vi "UI - By List.vi"(5 "Term (Methods)":string="Methods", 7 "Msg Chain":string, 8 "error in (no error)":errorcluster {"code" format="Error %.0f"}, 10 "UI Docs":refnum<class "GUI Documentation.lvclass">[](array[class]), 11 "VIDoc Printer - Confluence In":refnum<class "VIDoc Printer - Confluence.lvclass">) -> (0 "error out":errorcluster {"code" format="Error %.0f"}, 3 "VIDoc Printer - Confluence Out":refnum<class "VIDoc Printer - Confluence.lvclass">)   [LabVIEW 2023, in "VIDoc Printer - Confluence.lvlib" / "VIDoc Printer - Confluence.lvclass"]
uses:
  VIDoc Printer - Confluence.lvclass
  <vilib>/DMC/VIDoc/Framework/Parsing/GUI Documentation/GUI Documentation.lvclass
  Confluence Formatting/Types/Format Combo Box.ctl
  <vilib>/DMC/VIDoc/Framework/Printer/VIDoc Printer.lvclass/VIDoc Printer.ctl
  VIDoc Printer - Confluence.lvclass/VIDoc Printer - Confluence.ctl
  <vilib>/DMC/VIDoc/Framework/Parsing/GUI Documentation/GUI Documentation.lvclass/GUI Documentation.ctl
  Types/VI Method Types.ctl
  <vilib>/DMC/VIDoc/Framework/Printer/Accessors/Get VI Settings - List Detail Level.vi
  <vilib>/DMC/VIDoc/Framework/Parsing/GUI Documentation/Get VI Info.vi
  <vilib>/DMC/VIDoc/Framework/Printer/Accessors/Get Formatting Settings - Bookmark Options.vi
  Accessors/Get Sortable Tables.vi
  Accessors/Get Temporary Image Directory+.vi
  Accessors/Get VI By List Expand.vi
  <vilib>/Utility/libraryn.llb/Create Directory Recursive.vi
  Confluence Formatting/Confluence Formatting.lvlib
  <vilib>/DMC/VIDoc/Framework/Printer/VIDoc Printer.lvclass
  <vilib>/DMC/VIDoc/Framework/UI Interaction/Interface/UI Interaction.lvclass
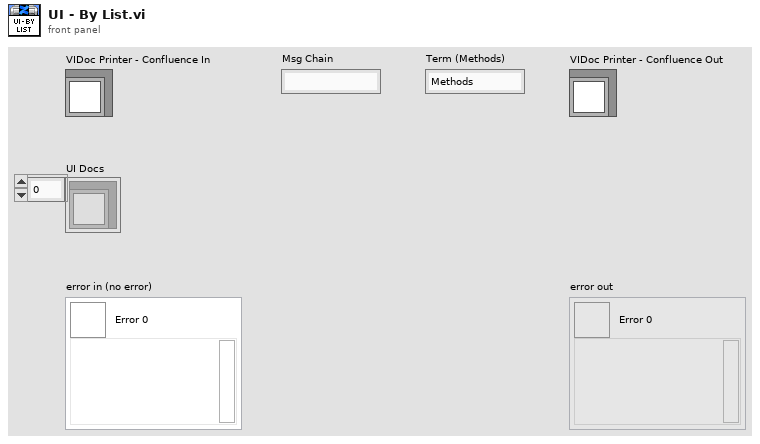
[diagram p1: front panel]
types:
  T1 = typedef "Confluence Formatting.lvlib/Format Combo Box.ctl" = string
  T2 = typedef "VIDoc Printer.lvlib/Printer Settings.lvclass/VI Settings.ctl" = cluster{"Memory":bool, "By Folder":bool, "By Tree":bool, "By List":bool, "Methods":bool, "Method Options":cluster{"Front Panels":bool, "Options":bool, "Controls":bool}, "List Detail Level":T3, "Methods Detail Level":T3, "Controls Detail Level":T3}
  T3 = typedef "VIDoc Printer.lvlib/Printer Settings.lvclass/Detail Level Enum.ctl" = enum16{"None", "Minimal", "Standard", "Full"}
  T4 = typedef "VIDoc Printer.lvlib/Printer Settings.lvclass/Bookmark Options.ctl" = cluster{"Bookmarks as New Line in VI Descriptions":bool, "Unique Bookmark Tags Only":bool, "Include Tag and Text":bool}
  T5 = typedef "VIDoc Printer - Confluence.lvlib/VIDoc Printer - Confluence.lvclass/VI Method Types.ctl" = enum16{"Library", "Class", "Interface", "LLB", "UI", "List"}
  T6 = typedef "VIDoc Parsing.lvlib/Method Spec Cluster.ctl" = cluster{"VI Type Ext":T7, "Name":string, "Path":path, "Get Conpane Image":T8, "Description":string, "Get Library Access Scope":enum32{"invalid scope", "public", "private", "protected", "community"}, "Dispatch":T9, "ContainsCompiledCode":bool, "Exec.IsReentrant":bool, "Exec.ReentrancyType":enum16{"Share clones between instances", "Preallocate clone for each instance"}, "ExecInlining":bool, "ExecInlineIfPossible":bool, "Auto Err Handling":bool, "CodeComplexity":sgl, "Bookmark Tags":string[], "Control VI Type":enum32{"not a control VI", "control", "typedef", "strict typedef"}, "Controls":T10[], "VI Type":enum32{"invalid VI type", "Standard VI", "Control VI", "Global VI", "Polymorphic VI", "Configuration VI", "SubSystem", "Facade VI", "Method VI", "Statechart Diagram VI"}, "Minimum Size":T12, "Front Panel Window:Title":string, "Front Panel Window:Behavior":enum32{"Invalid", "Default", "Floating", "Floating/Auto-Hide", "Modal"}, "Front Panel Window:Closeable":bool, "Must Override":bool, "Must Use Parent Implementation":bool, "VI Icon":T8, "Front Panel":T8, "History:Revision Number":u32, "Metrics:Total Data Size":u32, "Execution:Allow Debugging":bool, "Execution:Preferred Exec System":enum32{"invalid execution system", "user interface", "standard", "instrument i/o", "data acquisition", "other 1", "other 2", "same as caller"}, "Execution:Priority":enum32{"invalid priority", "background priority", "normal priority", "above normal priority", "high priority", "time critical priority", "subroutine"}, "BM Tag Text":string[], "Block Diagram":T8, "Structure Tree":T13[]}
  T7 = typedef "VIDoc Parsing.lvlib/VI Type Extended Enum.ctl" = enum16{"Unknown", "Class Method", "Class Accessor Get", "Class Accessor Set", "Class Control", "Library Method", "Library Control", "VI", "Control"}
  T8 = typedef "imagedata.ctl" = cluster{"image type":i32, "image depth":i32, "image":u8[], "mask":u8[], "colors":u32[], "Rectangle":cluster{"left":i16, "top":i16, "right":i16, "bottom":i16}}
  T9 = typedef "VIDoc Parsing.lvlib/Class Dispatch Type Enum.ctl" = enum16{"None", "Static", "Dynamic"}
  T10 = typedef "VIDoc Parsing.lvlib/Controls Info Cluster.ctl" = cluster{"Name":string, "Description":string, "Data Type":string, "Tip Strip":string, "UID":i32, "Image Data":T8, "ToggleKeyBind":T11, "Raw Label":string, "Raw Caption":string}
  T11 = typedef "LVKeyTypeDef.ctl" = cluster{"Focus":bool, "Control":bool, "Shift":bool, "Key":string}
  T12 = typedef "LVPointTypeDef.ctl" = cluster{"Horizontal":i16, "Vertical":i16}
  T13 = typedef "VIDoc Parsing.lvlib/Structure Reporter.lvlib/Tree Cluster.ctl" = cluster{"Object Class Name":string, "Labels":string[], "Child Tag":string, "Item Indent":i32, "Child Only?":bool, "Glyph Index":i32}
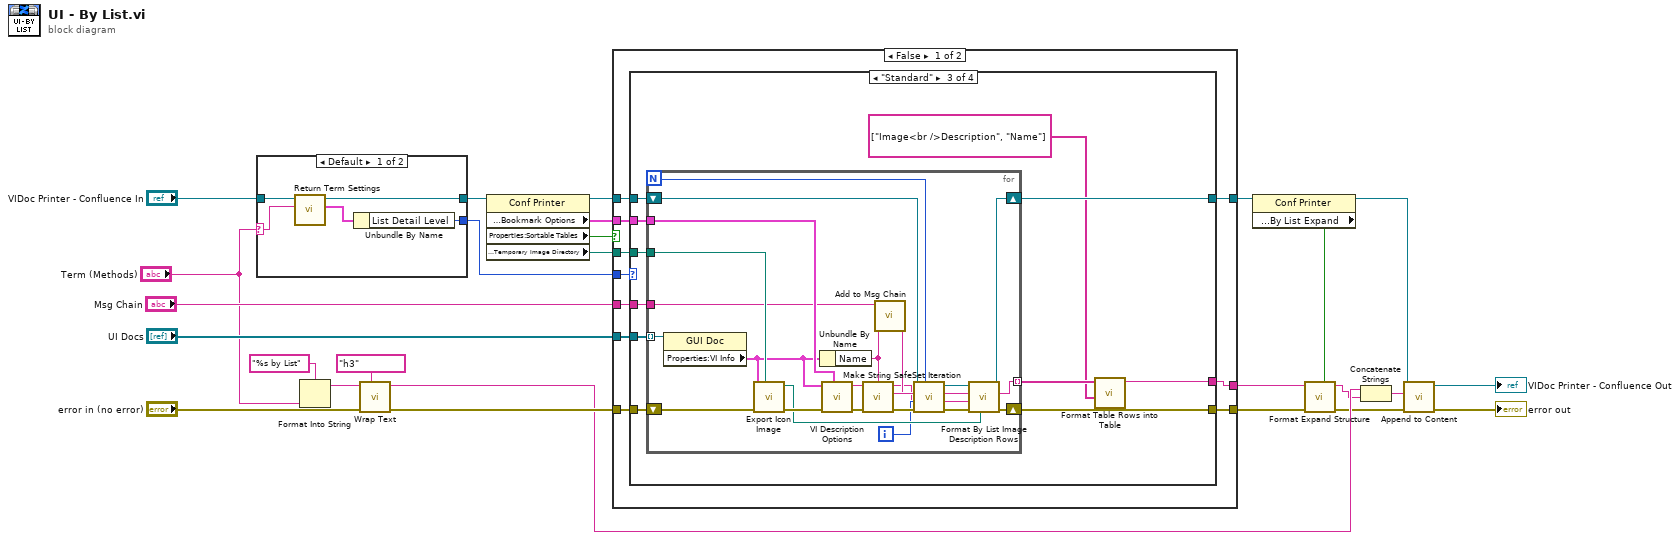
[diagram p0: block diagram]
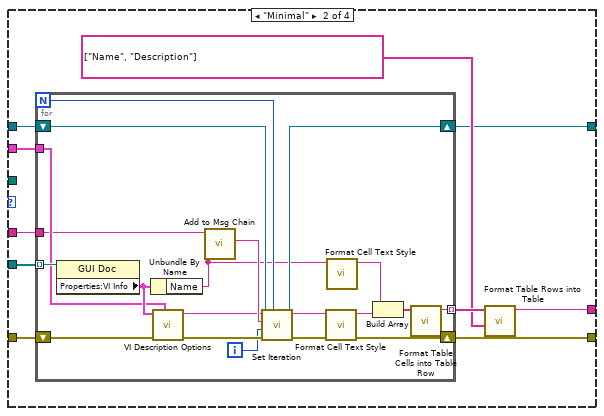
[diagram p3: hidden frame]
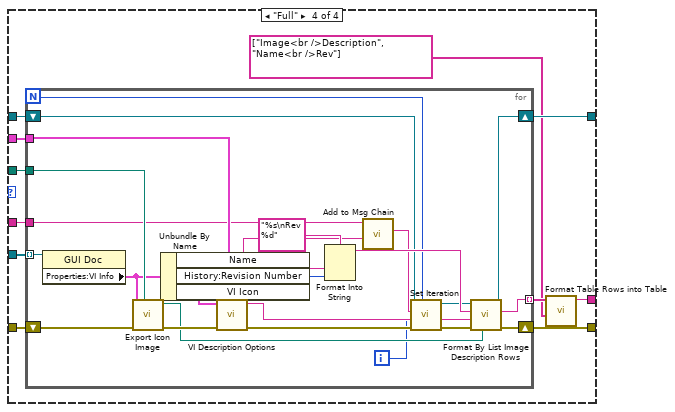
[diagram p4: hidden frame]
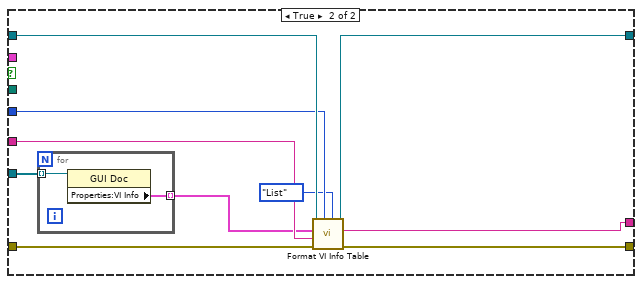
[diagram p5: hidden frame]
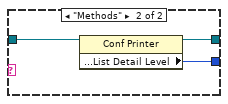
[diagram p6: hidden frame]
diagram:
  n1 = case shown="Default" "Term (Methods)" {
    selector: "Term (Methods)" -> [w29 _]
    tunnel: "VIDoc Printer - Confluence In" -> [w31 w34]
    tunnel: [w30 w33] -> w10
    tunnel: [w27 w32] -> w9
    frame Default {
      n2 = call <vilib>:"Return Term Settings.vi"("Term"=w29, "Printer in"=w31) -> ("Term Settings"=w28:T2, "Printer out"=w30:refnum<class "VIDoc Printer - Confluence.lvclass">)  [unwired: 6 in, 2 out]
      n3 = Unbundle By Name(w28) -> ("List Detail Level"=w27:T3)
    }
    frame "Methods" {
      n4 = property class="Conf Printer"(reference=w34) -> (reference out=w33:refnum<class "VIDoc Printer - Confluence.lvclass">, "Properties:Settings:VI Members:List Detail Level"=w32:T3)  [unwired: 1 in, 1 out]
    }
  }
  n5 = Format Into String(format string="%s by List", "Term (Methods)") -> (resulting string=w20:string)  [unwired: 2 in, 1 out]
  n6 = call "Wrap Text.vi"("Formatting"=T1 "h3", "Error in"="error in (no error)", "String"=w20) -> ("Error out"=w19:errorcluster, "Wrapped String"=w13:string)  [unwired: 7 in]
  n7 = property class="Conf Printer"(reference=w10) -> (reference out=w16:refnum<class "VIDoc Printer - Confluence.lvclass">, "Properties:Settings:Formatting Options:Bookmark Options"=w11:T4, "Properties:Sortable Tables"=w3:bool, "Properties:Temporary Image Directory"=w2:path)  [unwired: 1 in, 1 out]
  n8 = case shown="False" w3 {
    tunnel: w19 -> [w44 w150]
    tunnel: [w43 w149] -> w18
    tunnel: "UI Docs" -> [w42 w142]
    tunnel: w16 -> [w41 w147]
    tunnel: [w40 w146] -> w15
    tunnel: w2 -> [w39 _]
    tunnel: "Msg Chain" -> [w38 w143]
    tunnel: w11 -> [w37 _]
    tunnel: w9 -> [w36 w145]
    tunnel: [w35 w148] -> w7
    frame False {
      n9 = case shown="\"Standard\"" w36 {
        tunnel: w44 -> [w46 w54 w83 w115]
        tunnel: [w46 w51 w77 w109] -> w43
        tunnel: w42 -> [_ w56 w85 w117]
        tunnel: w37 -> [_ w55 w84 w116]
        tunnel: [_ w52 w79 w111] -> w35
        tunnel: w41 -> [w45 w49 w81 w113]
        tunnel: [w45 w48 w80 w112] -> w40
        tunnel: w39 -> [_ _ w82 w114]
        tunnel: w38 -> [_ w47 w75 w107]
        frame "None", Default {
        }
        frame "Minimal" {
          n10 = for {
            N -> [w64]
            tunnel: w56 -> [w74] mode=indexing
            tunnel: w55 -> [w72]
            shift-right: [w67] -> w51
            shift-left: w54 -> [w71]
            tunnel: [w69] -> w53 mode=indexing
            shift-right: [w65] -> w48
            shift-left: w49 -> [w66]
            tunnel: w47 -> [w62]
            i -> [w63]
            n11 = property class="GUI Doc"(reference=w74) -> ("Properties:VI Info"=w73:T6)  [unwired: 1 in, 2 out]
            n12 = Unbundle By Name(w73) -> ("Name"=w59:string)
            n13 = call <vilib>:"VI Description Options.vi"("Bookmark Options"=w72, "Error in"=w71, "VI Info"=w73) -> ("Error out"=w68:errorcluster, "Description"=w58:string)  [unwired: 7 in]
            n14 = call <vilib>:"Add to Msg Chain.vi"("New"=w59, "Msg Chain in"=w62) -> ("Msg Chain out"=w61:string)  [unwired: 9 in]
            n15 = call <vilib>:"Set Iteration.vi"("Progress Max"=w64, "error in (no error)"=w68, "Progress Value"=w63, "Message (No Message Update)"=w61, "VIDoc Printer In"=w66) -> ("error out"=w67:errorcluster, "VIDoc Printer Out"=w65:refnum<class "VIDoc Printer - Confluence.lvclass">)  [unwired: 4 in, 1 out]
            n16 = call "Format Cell Text Style.vi"("String"=w58) -> ("Formatted Text"=w57:string)  [unwired: 9 in, 1 out]
            n17 = call "Format Cell Text Style.vi"("String"=w59) -> ("Formatted Text"=w60:string)  [unwired: 9 in, 1 out]
            n18 = Build Array(w60, w57) -> (w70:string[])
            n19 = call "Format Table Cells into Table Row.vi"("Table Cells"=w70) -> ("Table Row Text"=w69:string)  [unwired: 10 in]
          }
          n20 = call "Format Table Rows into Table.vi"("Table Headers"=string[] ["Name", "Description"], "Table Rows"=w53) -> ("Table Text"=w52:string)  [unwired: 9 in]
        }
        frame "Standard" {
          n21 = for {
            N -> [w91]
            tunnel: w85 -> [w106] mode=indexing
            tunnel: w84 -> [w105]
            shift-right: [w100] -> w77
            shift-left: w83 -> [w103]
            tunnel: w82 -> [w104]
            shift-right: [w99] -> w80
            shift-left: w81 -> [w93]
            tunnel: [w96] -> w78 mode=indexing
            tunnel: w75 -> [w89]
            i -> [w90]
            n22 = property class="GUI Doc"(reference=w106) -> ("Properties:VI Info"=w101:T6)  [unwired: 1 in, 2 out]
            n23 = call <vilib>:"Export Icon Image.vi"("Temporary Image Directory"=w104, "Error in"=w103, "VI Info"=w101) -> ("Error out"=w102:errorcluster, "Image Path"=w97:path)  [unwired: 7 in]
            n24 = Unbundle By Name(w101) -> ("Name"=w88:string)
            n25 = call <vilib>:"VI Description Options.vi"("Bookmark Options"=w105, "Error in"=w102, "VI Info"=w101) -> ("Error out"=w95:errorcluster, "Description"=w98:string)  [unwired: 7 in]
            n26 = call "Make String Safe.vi"("Raw String"=w98) -> ("String out"=w86:string)  [unwired: 9 in, 1 out]
            n27 = call <vilib>:"Add to Msg Chain.vi"("New"=w88, "Msg Chain in"=w89) -> ("Msg Chain out"=w87:string)  [unwired: 9 in]
            n28 = call <vilib>:"Set Iteration.vi"("Progress Max"=w91, "error in (no error)"=w95, "Progress Value"=w90, "Message (No Message Update)"=w87, "VIDoc Printer In"=w93) -> ("error out"=w94:errorcluster, "VIDoc Printer Out"=w92:refnum<class "VIDoc Printer - Confluence.lvclass">)  [unwired: 4 in, 1 out]
            n29 = call "Format By List Image Description Rows.vi"("Image"=w97, "error in (no error)"=w94, "Description"=w86, "Name"=w88, "VIDoc Printer - Confluence In"=w92) -> ("error out"=w100:errorcluster, "Table Rows Text"=w96:string, "VIDoc Printer - Confluence Out"=w99:refnum<class "VIDoc Printer - Confluence.lvclass">)  [unwired: 3 in, 1 out]
          }
          n30 = call "Format Table Rows into Table.vi"("Table Headers"=string[] ["Image<br />Description", "Name"], "Table Rows"=w78) -> ("Table Text"=w79:string)  [unwired: 9 in]
        }
        frame "Full" {
          n31 = for {
            N -> [w122]
            tunnel: w117 -> [w140] mode=indexing
            tunnel: w116 -> [w139]
            shift-right: [w134] -> w109
            shift-left: w115 -> [w137]
            tunnel: w114 -> [w138]
            shift-right: [w133] -> w112
            shift-left: w113 -> [w124]
            tunnel: [w130] -> w110 mode=indexing
            tunnel: w107 -> [w120]
            i -> [w121]
            n32 = property class="GUI Doc"(reference=w140) -> ("Properties:VI Info"=w135:T6)  [unwired: 1 in, 2 out]
            n33 = call <vilib>:"Export Icon Image.vi"("Temporary Image Directory"=w138, "Error in"=w137, "VI Info"=w135) -> ("Error out"=w136:errorcluster, "Image Path"=w131:path)  [unwired: 7 in]
            n34 = Unbundle By Name(w135) -> ("Name"=w119:string, "History:Revision Number"=w128:u32)  [unwired: 1 out]
            n35 = call <vilib>:"VI Description Options.vi"("Bookmark Options"=w139, "Error in"=w136, "VI Info"=w135) -> ("Error out"=w126:errorcluster, "Description"=w132:string)  [unwired: 7 in]
            n36 = Format Into String(format string="%s\nRev %d", w119, w128) -> (resulting string=w127:string)  [unwired: 2 in, 1 out]
            n37 = call <vilib>:"Add to Msg Chain.vi"("New"=w119, "Msg Chain in"=w120) -> ("Msg Chain out"=w118:string)  [unwired: 9 in]
            n38 = call <vilib>:"Set Iteration.vi"("Progress Max"=w122, "error in (no error)"=w126, "Progress Value"=w121, "Message (No Message Update)"=w118, "VIDoc Printer In"=w124) -> ("error out"=w125:errorcluster, "VIDoc Printer Out"=w123:refnum<class "VIDoc Printer - Confluence.lvclass">)  [unwired: 4 in, 1 out]
            n39 = call "Format By List Image Description Rows.vi"("Image"=w131, "error in (no error)"=w125, "Description"=w132, "Name"=w127, "VIDoc Printer - Confluence In"=w123) -> ("error out"=w134:errorcluster, "Table Rows Text"=w130:string, "VIDoc Printer - Confluence Out"=w133:refnum<class "VIDoc Printer - Confluence.lvclass">)  [unwired: 3 in, 1 out]
          }
          n40 = call "Format Table Rows into Table.vi"("Table Headers"=string[] ["Image<br />Description", "Name<br />Rev"], "Table Rows"=w110) -> ("Table Text"=w111:string)  [unwired: 9 in]
        }
      }
    }
    frame True {
      n41 = for {
        tunnel: w142 -> [w152] mode=indexing
        tunnel: [w151] -> w141 mode=indexing
        n42 = property class="GUI Doc"(reference=w152) -> ("Properties:VI Info"=w151:T6)  [unwired: 1 in, 2 out]
      }
      n43 = call "Format VI Info Table.vi"("Type"=VI_Method_Types."List", "Methods"=w145, "Error in"=w150, "Msg Chain"=w143, "VI Info Array"=w141, "VIDoc Printer - Confluence In"=w147) -> ("Error out"=w149:errorcluster, "Table String"=w148:string, "VIDoc Printer - Confluence Out"=w146:refnum<class "VIDoc Printer - Confluence.lvclass">)  [unwired: 3 in]
    }
  }
  n44 = property class="Conf Printer"(reference=w15) -> (reference out=w5:refnum<class "VIDoc Printer - Confluence.lvclass">, "Properties:Expand?:VI:By List Expand"=w4:bool)  [unwired: 1 in, 1 out]
  n45 = call "Format Expand Structure.vi"("Enable? (T)"=w4, "Error in"=w18, "Content"=w7) -> ("Error out"=w8:errorcluster, "Expand String"=w6:string)  [unwired: 7 in]
  n46 = Concatenate Strings(w13, w6) -> (w14:string)
  n47 = call "Append to Content.vi"("error in (no error)"=w8, "Content"=w14, "VIDoc Printer - Confluence In"=w5) -> ("error out"=→"error out":errorcluster, "VIDoc Printer - Confluence Out"=→"VIDoc Printer - Confluence Out":refnum<class "VIDoc Printer - Confluence.lvclass">)  [unwired: 7 in]
